vi "Check If Initialised.vi"(8 "error in (no error)":errorcluster, 11 "Session in":refnum<class "Session.lvclass">) -> (0 "error out":errorcluster, 2 "Initialised":bool, 3 "Session out":refnum<class "Session.lvclass">)   [LabVIEW 2020, in "CTI.lvlib" / "Session.lvclass"]
doc: "Acquires the DeviceComm instance that is used to interact with a device. This VI can be used by connection wrapper classes and peripheral classes to safely perform a handful of device operations without being interrupted by other parallel loops. Be sure to return the DeviceComms instance by calling <b>Return DeviceComms.vi</b> otherwise the session will fail to perform as expected and future attempts to interact with the device will fail."
uses:
  Session.lvclass
  Session.lvclass/Session.ctl
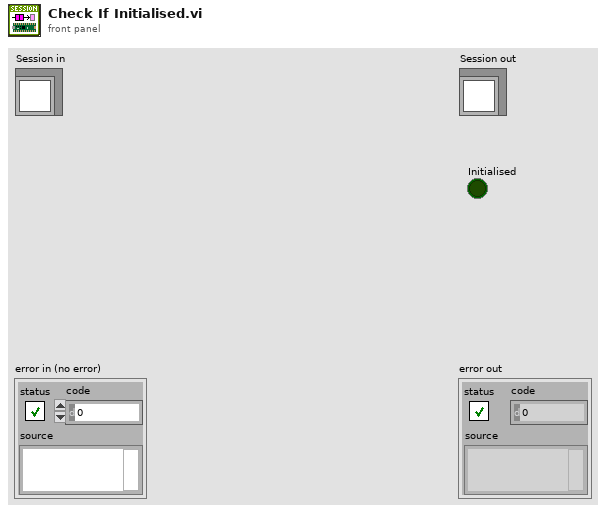
[diagram p1: front panel]
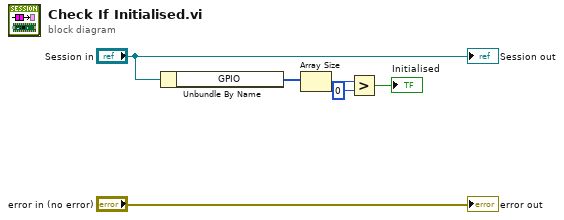
[diagram p0: block diagram]
diagram:
  n1 = Unbundle By Name("Session in") -> ("GPIO"=w4:u8[])
  n2 = Array Size(array=w4) -> (size(s)=w3:i32)
  n3 = Greater?(x=w3, y=0) -> (0:→"Initialised":bool)
  "error out" <- "error in (no error)"
  "Session out" <- "Session in"
